vi "addEdge.vi"(0 "reference":refnum<class "NoteNode.lvclass">, 1 "egde":refnum<class "AbstractEdge.lvclass">, 2 "p1":T1 {"y" format="%.2f"; "x" format="%.2f"}, 3 "p2":T1 {"y" format="%.2f"; "x" format="%.2f"}, 5 "error in (no error)":errorcluster) -> (14 "reference out":refnum<class "NoteNode.lvclass">, 15 "edgeHasEndNode":bool, 19 "error out":errorcluster)   [LabVIEW 2020, in "NoteNode.lvclass"]
doc: "public boolean addEdge(Edge e, Point2D p1, Point2D p2)"
uses:
  <resource>/Framework/Providers/Open_GDS/UML/NoteNode_class/NoteNode.lvclass
  C:/Program Files (x86)/National Instruments/LabVIEW 2020/resource/Framework/Providers/Open_GDS/UML/RectangularNode_class/RectangularNode.lvclass
  C:/Program Files (x86)/National Instruments/LabVIEW 2020/resource/Framework/Providers/Open_GDS/UML/AbstractNode_class/AbstractNode.lvclass
  <resource>/Framework/Providers/Open_GDS/UML/AbstractEdge_class/AbstractEdge.lvclass
  <resource>/Framework/Providers/Open_GDS/UML/General/Point/Point Point2D.ctl
  <resource>/Framework/Providers/Open_GDS/UML/PointNode_class/PointNode.lvclass
  <resource>/Framework/Providers/Open_GDS/UML/RectangularNode_class/RectangularNode.lvclass
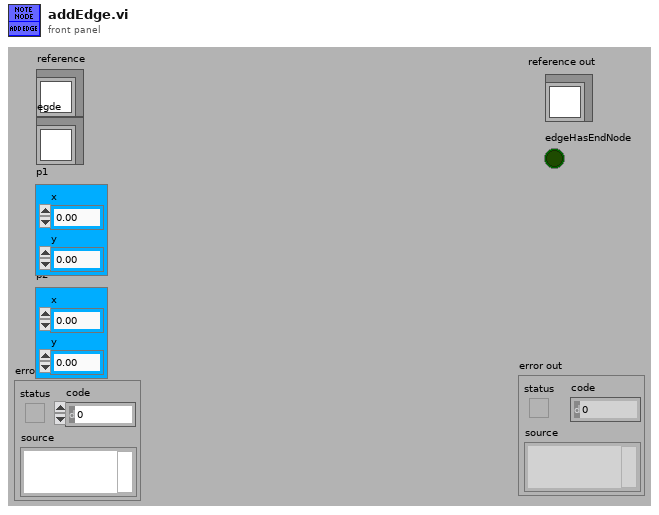
[diagram p1: front panel]
types:
  T1 = typedef "Point Point2D.ctl" = cluster{"x":dbl, "y":dbl}
  T2 = typedef "RectangularNode.lvclass/ObjectAttributes.ctl" = cluster{"bounds":T3}
  T3 = typedef "Rectangle Rectangle2D.ctl" = cluster{"x":dbl, "y":dbl, "width":dbl, "height":dbl}
  T4 = typedef "NoteNode.lvclass/ObjectAttributes.ctl" = cluster{"DEFAULT_WIDTH":i32, "DEFAULT_HEIGHT":i32, "DEFAULT_COLOR":u32, "FOLD_X":i32, "FOLD_Y":i32, "color":u32, "text":refnum<class "MultiLineString.lvclass">, "pointNodes":refnum<class "AbstractNode.lvclass">[]}
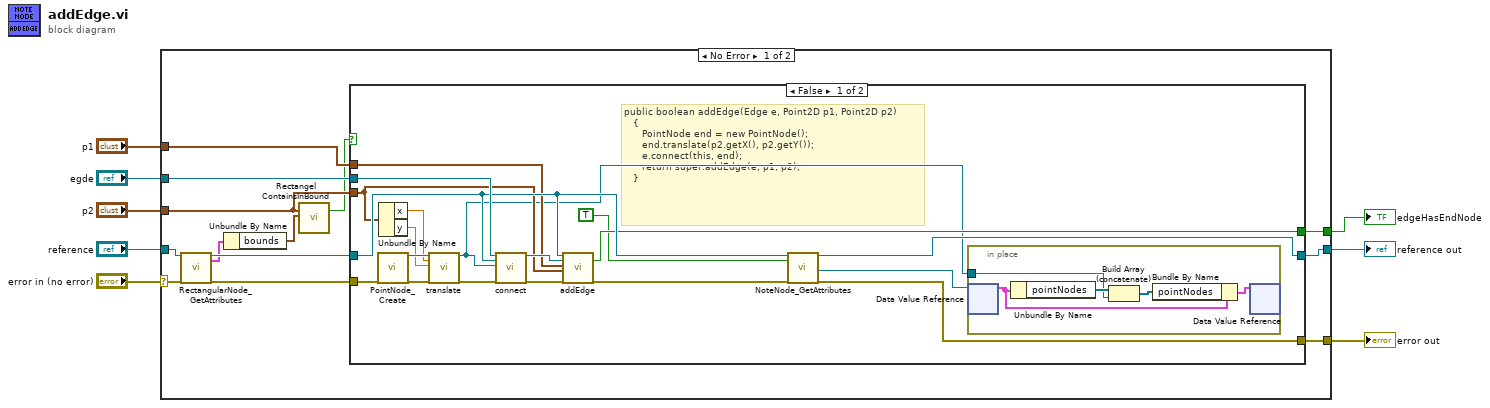
[diagram p0: block diagram]
diagram:
  n1 = case shown="No Error" "error in (no error)" {
    selector: "error in (no error)" -> [w18 w48]
    tunnel: "reference" -> [w21 w49]
    tunnel: [w20 w48] -> w7
    tunnel: [w19 w49] -> w6
    tunnel: "egde" -> [w17 _]
    tunnel: "p1" -> [w16 _]
    tunnel: "p2" -> [w15 _]
    tunnel: [w10 _] -> w1
    frame No Error {
      n2 = call <resource>:"RectangularNode_GetAttributes.vi"("reference in"=w21, "error in (no error)"=w18) -> ("reference out"=w14:refnum<class "NoteNode.lvclass">, "Data"=w9:T2, "error out"=w13:errorcluster)  [unwired: 14 in, 1 out]
      n3 = Unbundle By Name(w9) -> ("bounds"=w12:T3)
      n4 = call <resource>:"Rectangel ContainsInBound.vi"("point2D"=w15, "bounds"=w12) -> ("contains"=w11:bool)  [unwired: 2 in, 15 out]
      n5 = case shown="False" w11 {
        tunnel: w17 -> [w40 _]
        tunnel: w16 -> [w28 _]
        tunnel: [w34 w47] -> w19
        tunnel: [w33 w46] -> w20
        tunnel: w14 -> [w31 w47]
        tunnel: w13 -> [w32 w46]
        tunnel: w15 -> [w27 _]
        tunnel: [w25 _] -> w10
        frame False {
          # "public boolean addEdge(Edge e, Point2D p1, Point2D p2)\n   {\n      PointNode end = new PointNode();\n      end.translate(p2.getX(), p2.getY());\n      e.connect(this, end);\n      return super.addEdge(e, p1, p2);\n   }"
          n6 = call <resource>:"PointNode_Create.vi"("error in (no error)"=w32) -> ("reference out"=w39:refnum<class "PointNode.lvclass">, "error out"=w38:errorcluster)  [unwired: 1 in, 16 out]
          n7 = Unbundle By Name(w27) -> ("x"=w37:dbl, "y"=w36:dbl)
          n8 = call-dynamic "translate.vi"("reference"=w39, "dx"=w37, "dy"=w36, "error in (no error)"=w38) -> ("reference out"=w22:refnum<class "PointNode.lvclass">, "error out"=w35:errorcluster)  [unwired: 14 in]
          n9 = call-dynamic "connect.vi"("reference"=w40, "startNode"=w31, "endNode"=w22, "error in (no error)"=w35) -> ("reference out"=w29:refnum<class "AbstractEdge.lvclass">, "error out"=w30:errorcluster)  [unwired: 14 in]
          n10 = call-parent "addEdge.vi"("reference"=w31, "egde"=w29, "p1"=w28, "p2"=w27, "error in (no error)"=w30) -> ("edgeHasEndNode"=w25:bool, "error out"=w26:errorcluster)  [unwired: 12 in, 1 out]
          n11 = call <resource>:"NoteNode_GetAttributes.vi"("reference in"=w31, "OnlyGetDvrReference(False)"=TRUE, "error in (no error)"=w26) -> ("reference out"=w34:refnum<class "NoteNode.lvclass">, "DataRef"=w23:refnum<data-value>, "error out"=w33:errorcluster)  [unwired: 13 in, 1 out]
          n12 = in-place {
            in-place-border: w22 -> [w41]
            n13 = in-place-dvr #1(w23) -> (w45:T4)  [unwired: 1 out]
            n14 = Unbundle By Name(w45) -> ("pointNodes"=w42:refnum<class "AbstractNode.lvclass">[])
            n15 = Build Array (concatenate)(w42, w41) -> (w44:refnum<class "AbstractNode.lvclass">[])
            n16 = Bundle By Name(cluster=w45, "pointNodes"=w44) -> (w43:T4)
            n17 = in-place-dvr #1(w43) -> ()  [unwired: 2 out]
          }
        }
        frame True {
        }
      }
    }
    frame Error {
    }
  }
  "reference out" <- w6
  "error out" <- w7
  "edgeHasEndNode" <- w1
